vi "GetPosition.vi"(8 "error in (no error)":errorcluster, 11 "Window in":refnum<class "Window.lvclass">) -> (0 "error out":errorcluster, 2 "Window Position":cluster{"x":i32, "y":i32}, 3 "Window out":refnum<class "Window.lvclass">)   [LabVIEW 2020, in "GLF.lvlib" / "Window.lvclass"]
uses:
  Window.lvclass
  Window.lvclass/Window.ctl
  <vilib>/Saukko/LV SDL3/Sources/SDL3/Video/Video.lvlib
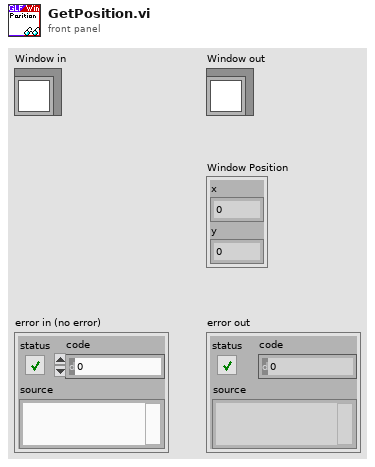
[diagram p1: front panel]
types:
  T1 = typedef "SDL3.lvlib/Video.lvlib/SDL_Window--pointer.ctl" = i64
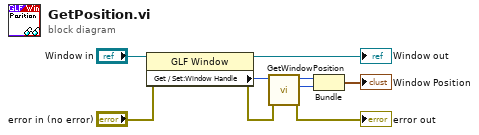
[diagram p0: block diagram]
diagram:
  n1 = property class="GLF Window"(reference="Window in", error in="error in (no error)") -> (reference out=→"Window out":refnum<class "Window.lvclass">, error out=w2:errorcluster, "Get / Set:Window Handle"=w1:T1)
  n2 = call <vilib>:"GetWindowPosition.vi"("No Error"=w2, "Window [SDL_Window *]"=w1) -> ("Error Out"=→"error out":errorcluster, "y"=w6:i32, "x"=w7:i32)  [unwired: 7 in]
  n3 = Bundle("x"=w7, "y"=w6) -> (→"Window Position":cluster{"x":i32, "y":i32})  [unwired: 1 in]
